vi "ASCII to hex.vi"(11 "ASCII string":string) -> (3 "hex string":string)   [LabVIEW 2015, in "Lengmur_socket.lvlib"]
uses:
  Lengmur_socket.lvlib
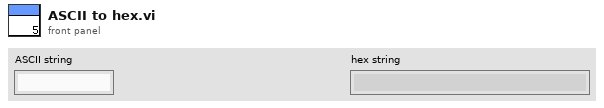
[diagram p1: front panel]
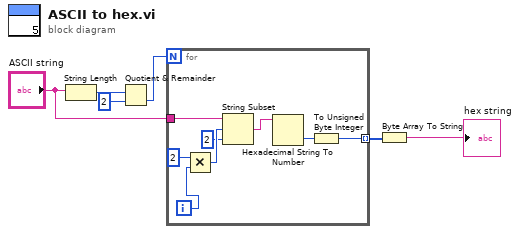
[diagram p0: block diagram]
diagram:
  n1 = String Length(string="ASCII string") -> (length=w5:i32)
  n2 = Quotient & Remainder(x=w5, y=2) -> (floor(x/y)=w4:i32)  [unwired: 1 out]
  n3 = for {
    N: w4 -> [_]
    tunnel: "ASCII string" -> [w14]
    tunnel: [w7] -> w2 mode=indexing
    i -> [w12]
    n4 = Multiply(x=2, y=w12) -> (x*y=w13:i32)
    n5 = String Subset(string=w14, offset (0)=w13, length (rest)=2 ("length (rest)")) -> (substring=w9:string)
    n6 = Hexadecimal String To Number(string=w9) -> (number=w8:u32)  [unwired: 2 in, 1 out]
    n7 = To Unsigned Byte Integer(number=w8) -> (unsigned 8bit integer=w7:u8)
  }
  n8 = Byte Array To String(unsigned byte array=w2) -> (string=→"hex string":string)
